vi "Test_IOVariable.vi"(8 "error in (no error)":errorcluster) -> (0 "error out":errorcluster)   [LabVIEW 2013]
uses:
  source/uri/URI.lvclass/URI.ctl
  source/components/path/URI-Component.Path.lvclass/URI-Component.Path.ctl
  source/components/path/URI-Component.Path.lvclass
  source/uri/Read scheme.vi
  source/uri/Read host.vi
  source/uri/Read path.vi
  source/uri/Read path segments.vi
  source/components/path/Get Segments.vi
  <vilib>/addons/_JKI Toolkits/Caraya/classes/Assert/Assert Equal Value_Variant.vi
  source/components/path/Get path (absolute).vi
  <vilib>/addons/_JKI Toolkits/Caraya/classes/Test/Test.lvclass
  <vilib>/addons/_JKI Toolkits/Caraya/classes/Assert/Assert.lvclass
  source/uri/URI.lvclass
  source/openURI.lvlib
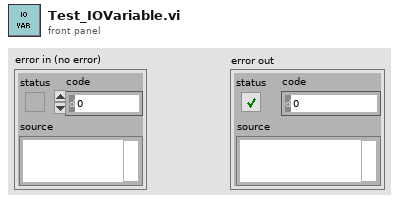
[diagram p1: front panel]
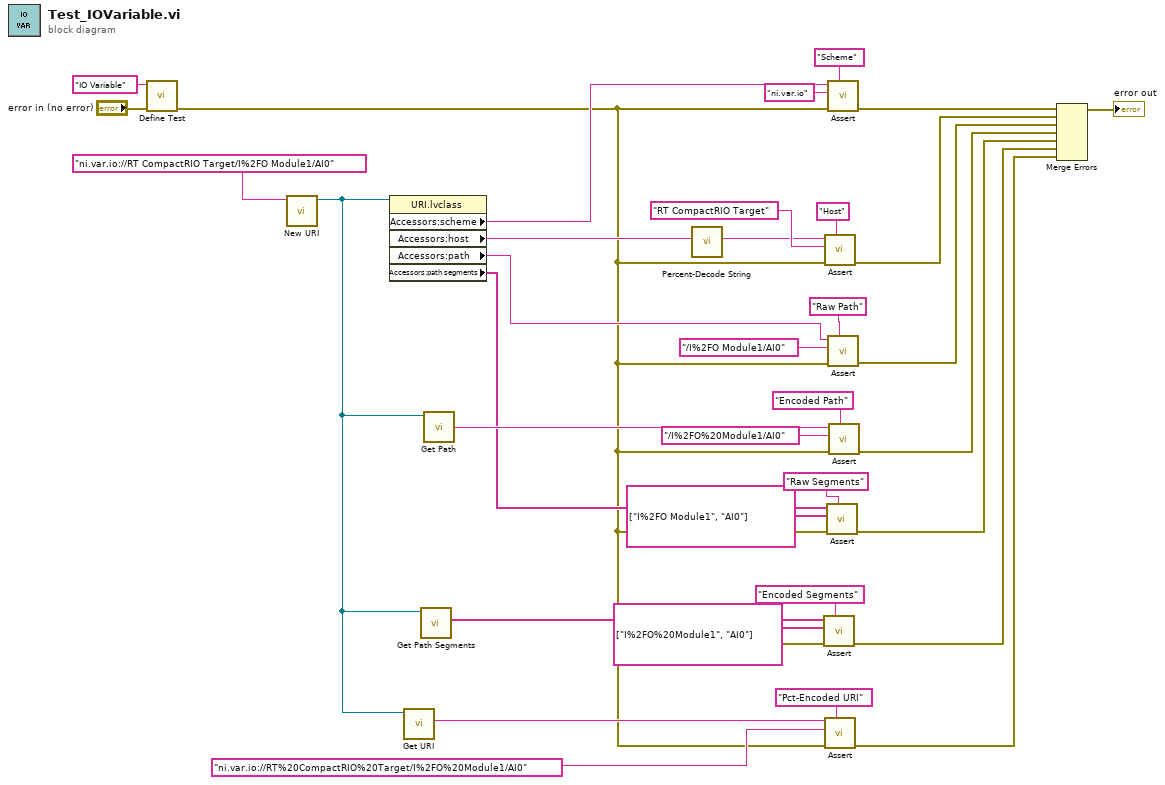
[diagram p0: block diagram]
diagram:
  n1 = call <vilib>:"Define Test.vi"("error in (no error)"="error in (no error)", "Label (VI Title)"="IO Variable") -> ("error out"=w1:errorcluster)  [unwired: 8 in, 1 out]
  n2 = call "New URI.vi"("URI"="ni.var.io://RT CompactRIO Target/I%2FO Module1/AI0") -> ("URI"=w2:refnum<class "URI.lvclass">)  [unwired: 9 in, 1 out]
  n3 = property on="Property Node" class="URI.lvclass"(reference=w2) -> ("Accessors:scheme"=w30:string, "Accessors:host"=w16:string, "Accessors:path"=w14:string, "Accessors:path segments"=w3:string[])  [unwired: 1 in, 2 out]
  n4 = call "Get URI.vi"("URI in"=w2) -> ("URI String"=w12:string)  [unwired: 8 in, 2 out]
  n5 = call "Get Path Segments.vi"("URI in"=w2) -> ("Segments"=w5:string[])  [unwired: 8 in, 2 out]
  n6 = call "Get Path.vi"("URI in"=w2) -> ("path"=w6:string)  [unwired: 8 in, 2 out]
  n7 = call "Percent-Decode String.vi"("Pct-Encoded String"=w16) -> ("String"=w15:string)  [unwired: 10 in]
  n8 = call-poly <vilib>:"Assert.vi"("Label"="Encoded Segments" ("URI"), "error in (no error)"=w1, "Y"=string[] ["I%2FO%20Module1", "AI0"] ("Segments"), "X"=w5) -> ("error out"=w18:errorcluster)  [unwired: 6 in, 1 out]
  n9 = call-poly <vilib>:"Assert.vi"("Label"="Host" ("URI"), "error in (no error)"=w1, "Y"="RT CompactRIO Target" ("URI"), "X"=w15) -> ("error out"=w26:errorcluster)  [unwired: 6 in, 1 out]
  n10 = call-poly <vilib>:"Assert.vi"("Label"="Pct-Encoded URI" ("URI"), "error in (no error)"=w1, "Y"="ni.var.io://RT%20CompactRIO%20Target/I%2FO%20Module1/AI0" ("URI"), "X"=w12) -> ("error out"=w11:errorcluster)  [unwired: 6 in, 1 out]
  n11 = call-poly <vilib>:"Assert.vi"("Label"="Raw Segments" ("URI"), "error in (no error)"=w1, "Y"=string[] ["I%2FO Module1", "AI0"] ("Segments"), "X"=w3) -> ("error out"=w20:errorcluster)  [unwired: 6 in, 1 out]
  n12 = call-poly <vilib>:"Assert.vi"("Label"="Scheme" ("URI"), "error in (no error)"=w1, "Y"="ni.var.io" ("URI"), "X"=w30) -> ("error out"=w27:errorcluster)  [unwired: 6 in, 1 out]
  n13 = call-poly <vilib>:"Assert.vi"("Label"="Raw Path" ("URI"), "error in (no error)"=w1, "Y"="/I%2FO Module1/AI0" ("URI"), "X"=w14) -> ("error out"=w23:errorcluster)  [unwired: 6 in, 1 out]
  n14 = call-poly <vilib>:"Assert.vi"("Label"="Encoded Path" ("URI"), "error in (no error)"=w1, "Y"="/I%2FO%20Module1/AI0" ("URI"), "X"=w6) -> ("error out"=w7:errorcluster)  [unwired: 6 in, 1 out]
  n15 = Merge Errors(w27, w26, w23, w7, w20, w18, w11) -> (→"error out":errorcluster)
